vi "Disconnect.vi"(8 "error in (no error)":errorcluster) -> (3 "OUT":i32)   [LabVIEW 2017, in "HID_ARZ.lvlib"]
doc: "DISCONNECT Disconnect;"
uses:
  HID_ARZ.lvlib
  <userlib>/HID_ARZ/mcHID.dll
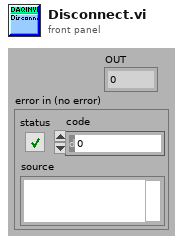
[diagram p1: front panel]
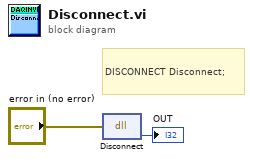
[diagram p0: block diagram]
diagram:
  # "DISCONNECT Disconnect;"
  n1 = dll-call lib="C:/Program Files (x86)/National Instruments/LabVIEW 2017/user.lib/HID_ARZ/mcHID.dll" fn="Disconnect"(error in="error in (no error)") -> ("return type"=→"OUT":i32)  [unwired: 2 in, 2 out]
